vi "Eval_SglVar_SglRes.vi"(8 "error in (no error)":errorcluster, 9 "varValue":dbl format="%#_13g", 11 "muExpr in":refnum<class "mupExpr.lvclass">) -> (0 "error out":errorcluster, 2 "Result":dbl, 3 "muExpr out":refnum<class "mupExpr.lvclass">)   [LabVIEW 2018, in "mupExpr.lvclass"]
doc: "Updates the value of the selected single variable then evaluates the expression.\nReturns a single result.\n\nIf multiple expressions have been input, the result of the last one in the list is returned.\n\nIf the variables are defined for bulk mode evaluation, only the first set (index 0) will be evaluated."
uses:
  mupExpr.lvclass
  mupExpr.lvclass/mupExpr.ctl
  mupLib/mupCheckError.vi
  <vilib>/Utility/error.llb/Error Cluster From Error Code.vi
  mupLib/mupLib.lvlib
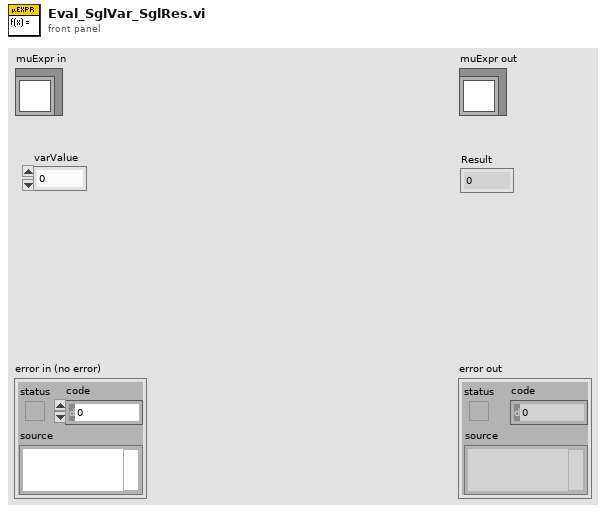
[diagram p1: front panel]
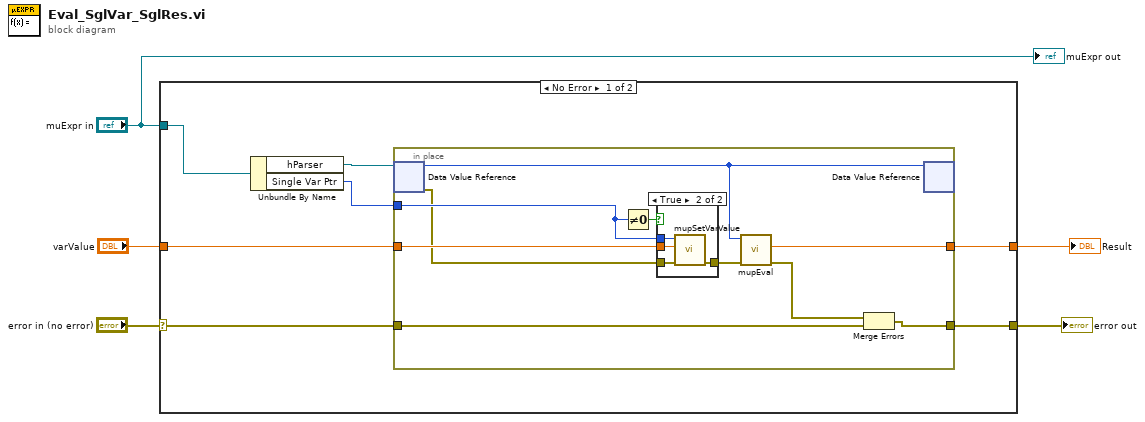
[diagram p0: block diagram]
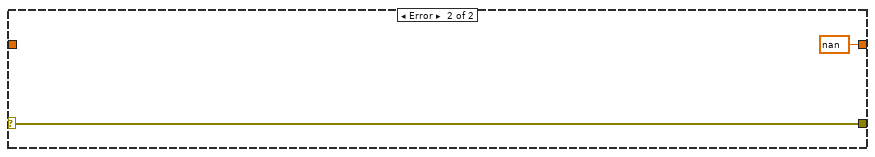
[diagram p3: hidden frame]
diagram:
  n1 = case shown="No Error" "error in (no error)" {
    selector: "error in (no error)" -> [w6 w29]
    tunnel: [w12 w29] -> w5
    tunnel: "muExpr in" -> [w11 _]
    tunnel: "varValue" -> [w10 _]
    tunnel: [w9 nan ("result")] -> w2
    frame No Error {
      n2 = Unbundle By Name(w11) -> ("hParser"=w8:refnum<data-value>, "Single Var Ptr"=w7:u64)
      n3 = in-place {
        in-place-border: w6 -> [w15]
        in-place-border: w10 -> [w22]
        in-place-border: [w14] -> w12
        in-place-border: [w21] -> w9
        in-place-border: w7 -> [w18]
        n4 = in-place-dvr #1(w8) -> (w17:u64, w13:errorcluster)
        n5 = Not Equal To 0?(x=w18) -> (x != 0?=w19:bool)
        n6 = case shown="True" w19 {
          tunnel: w13 -> [w23 w27]
          tunnel: w22 -> [_ w26]
          tunnel: [w23 w25] -> w20
          tunnel: w18 -> [_ w24]
          frame False {
          }
          frame True {
            n7 = call "mupSetVarValue.vi"("error in (no error)"=w27, "varValue"=w26, "varAddr in"=w24) -> ("error out"=w25:errorcluster)  [unwired: 7 in, 1 out]
          }
        }
        n8 = call "mupEval.vi"("error in (no error)"=w20, "hParser in"=w17) -> ("error out"=w16:errorcluster, "result"=w21:dbl)  [unwired: 7 in, 1 out]
        n9 = Merge Errors(w16, w15) -> (w14:errorcluster)
        n10 = in-place-dvr #1(w17) -> ()  [unwired: 2 out]
      }
    }
    frame Error {
    }
  }
  "error out" <- w5
  "Result" <- w2
  "muExpr out" <- "muExpr in"
